vi "Condition.vi"(8 "error in":errorcluster, 11 "Msg in":refnum<class "Msg.lvclass">) -> (0 "error out":errorcluster, 3 "Msg out":refnum<class "Msg.lvclass">)   [LabVIEW 2020, in "_Rescript.lvlib" / "Msg.lvlib" / "Msg.lvclass"]
uses:
  Msg.lvclass
  Msg.lvclass/Msg.ctl
  IO.ctl
  <vilib>/Utility/traverseref.llb/TRef Find Object By Label.vi
  _Shared/Name Specs/Name Specs.lvclass
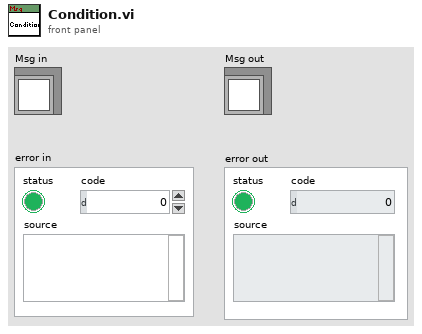
[diagram p1: front panel]
types:
  T1 = typedef "_Rescript.lvlib/Msg.lvlib/Msg.lvclass/IO.ctl" = enum16{"Input", "Output"}
  T2 = typedef "_Rescript.lvlib/Msg.lvlib/Msg.lvclass/Name.ctl" = cluster{"Name VI (Lib)":refnum<vi>, "Init Msg VI (Lib)":refnum<vi>, "Call VI (Lib)":refnum<vi>, "Recurse VI (Lib)":refnum<vi>, "Tell Self VI (Lib)":refnum<vi>, "Tell Parent VI (Lib)":refnum<vi>, "Tell Child VI (Lib)":refnum<vi>, "Tell Reply VI (Lib)":refnum<vi>}
  T3 = typedef "_Rescript.lvlib/Terminals.ctl" = set{i32}
  T4 = typedef "_Rescript.lvlib/Msg.lvlib/Msg.lvclass/Name Msg IO.ctl" = cluster{"PD Control (Class)":refnum<vi>, "PD Cluster (Class)":refnum<vi>, "Init Msg IO VI (Class)":refnum<vi>, "Read Msg IO VI (Class)":refnum<vi>, "Init Msg IO VI (Lib)":refnum<vi>, "Read Msg IO VI (Lib)":refnum<vi>, "Terminal Attributes (Init)":T5, "Terminal Attributes (Read)":T5}
  T5 = typedef "_Rescript.lvlib/Terminal Attributes.ctl" = map{i32, T6}
  T6 = typedef "_Rescript.lvlib/Attributes.ctl" = cluster{"Control":refnum<vi>, "Wire Rule":enum16{"Invalid Wire Rule", "Required", "Recommended", "Optional", "Dynamic Dispatch"}}
  T7 = typedef "_Shared.lvlib/Name Stuff.ctl" = cluster{"Type (Enum)":T8, "Type (String)":string, "Name Library File Path":path, "Name":string, "Name Type":string}
  T8 = typedef "_Shared.lvlib/Type.ctl" = enum16{"Actor", "Msg"}
  T9 = typedef "_Rescript.lvlib/Msg.lvlib/Msg.lvclass/Name Msg.ctl" = cluster{"Execute VI (Class)":refnum<vi>}
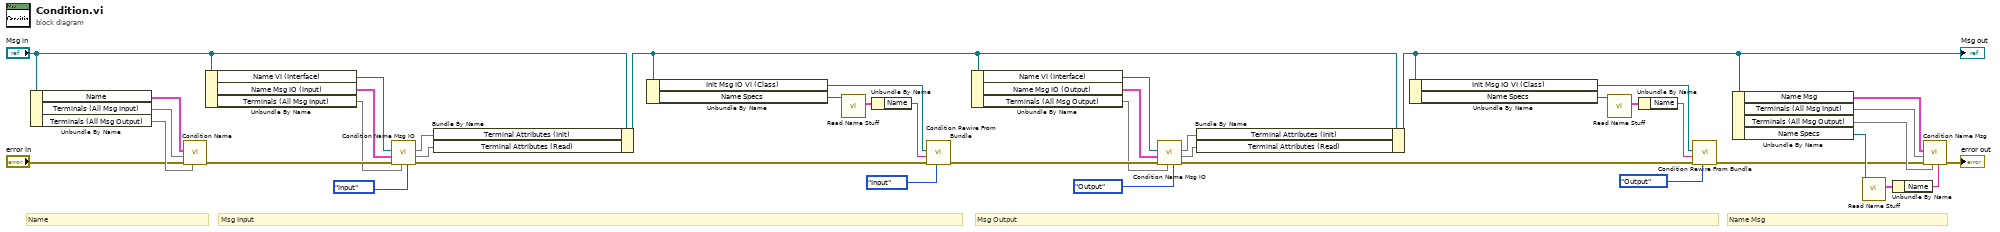
[diagram p0: block diagram]
diagram:
  # "Name Msg"
  # "Msg Output"
  # "Name"
  # "Msg Input"
  n1 = Unbundle By Name("Msg in") -> ("Name"=w40:T2, "Terminals (All Msg Input)"=w39:T3, "Terminals (All Msg Output)"=w38:T3)
  n2 = call "Condition Name.vi"("Terminals (All Msg Output)"=w38, "error in"="error in", "Terminals (All Msg Input)"=w39, "Name"=w40) -> ("error out"=w41:errorcluster)  [unwired: 7 in]
  n3 = Unbundle By Name("Msg in") -> ("Name VI (Interface)"=w33:refnum<vi>, "Name Msg IO (Input)"=w35:T4, "Terminals (All Msg Input)"=w4:T3)
  n4 = call "Condition Name Msg IO.vi"("IO"=IO."Input", "Terminals (All)"=w4, "error in"=w41, "Name Msg IO"=w35, "Name jettl Msg.Name VI (Interface)"=w33) -> ("error out"=w20:errorcluster, "Terminal Attributes (Read)"=w26:T5, "Terminal Attributes (Init)"=w25:T5)  [unwired: 4 in]
  n5 = Bundle By Name(cluster="Msg in", "Terminal Attributes (Init)"=w25, "Terminal Attributes (Read)"=w26) -> (w5:refnum<class "Msg.lvclass">)
  n6 = Unbundle By Name(w5) -> ("Init Msg IO VI (Class)"=w21:refnum<vi>, "Name Specs"=w24:refnum<class "Name Specs.lvclass">)
  n7 = call "Read Name Stuff.vi"("Name Specs in"=w24) -> ("Name Stuff"=w23:T7)  [unwired: 10 in]
  n8 = Unbundle By Name(w23) -> ("Name"=w22:string)
  n9 = call "Condition Rewire From Bundle.vi"("IO"=IO."Input", "error in"=w20, "Name"=w22, "VI?"=w21) -> ("error out"=w9:errorcluster)  [unwired: 7 in]
  n10 = Unbundle By Name(w5) -> ("Name VI (Interface)"=w17:refnum<vi>, "Name Msg IO (Output)"=w18:T4, "Terminals (All Msg Output)"=w3:T3)
  n11 = call "Condition Name Msg IO.vi"("IO"=IO."Output", "Terminals (All)"=w3, "error in"=w9, "Name Msg IO"=w18, "Name jettl Msg.Name VI (Interface)"=w17) -> ("error out"=w10:errorcluster, "Terminal Attributes (Read)"=w16:T5, "Terminal Attributes (Init)"=w15:T5)  [unwired: 4 in]
  n12 = Bundle By Name(cluster=w5, "Terminal Attributes (Init)"=w15, "Terminal Attributes (Read)"=w16) -> (w6:refnum<class "Msg.lvclass">)
  "Msg out" <- w6
  n13 = Unbundle By Name(w6) -> ("Init Msg IO VI (Class)"=w11:refnum<vi>, "Name Specs"=w14:refnum<class "Name Specs.lvclass">)
  n14 = call "Read Name Stuff.vi"("Name Specs in"=w14) -> ("Name Stuff"=w13:T7)  [unwired: 10 in]
  n15 = Unbundle By Name(w13) -> ("Name"=w12:string)
  n16 = call "Condition Rewire From Bundle.vi"("IO"=IO."Output", "error in"=w10, "Name"=w12, "VI?"=w11) -> ("error out"=w8:errorcluster)  [unwired: 7 in]
  n17 = Unbundle By Name(w6) -> ("Name Msg"=w30:T9, "Terminals (All Msg Input)"=w27:T3, "Terminals (All Msg Output)"=w28:T3, "Name Specs"=w36:refnum<class "Name Specs.lvclass">)
  n18 = call "Read Name Stuff.vi"("Name Specs in"=w36) -> ("Name Stuff"=w37:T7)  [unwired: 10 in]
  n19 = Unbundle By Name(w37) -> ("Name"=w29:string)
  n20 = call "Condition Name Msg.vi"("Name"=w29, "Terminals (All Msg Output)"=w28, "error in"=w8, "Terminals (All Msg Input)"=w27, "Name Msg"=w30) -> ("error out"=→"error out":errorcluster)  [unwired: 6 in]
